vi "Connect If Necessary.vi"(8 "error in (no error)":errorcluster, 11 "Plugin in":refnum<class "Modbus.lvclass">) -> (0 "error out":errorcluster, 3 "Plugin out":refnum<class "Modbus.lvclass">)   [LabVIEW 2026, in "Modbus.lvlib" / "Modbus.lvclass"]
uses:
  Modbus.lvclass
  Modbus.lvclass/Modbus.ctl
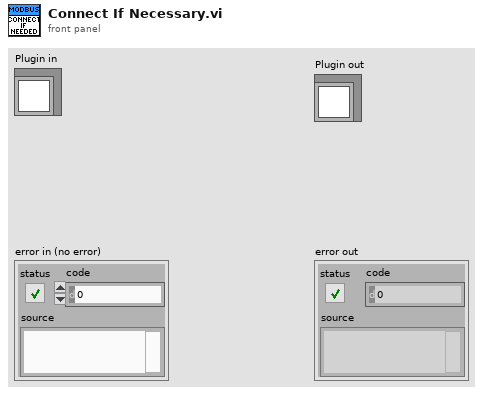
[diagram p1: front panel]
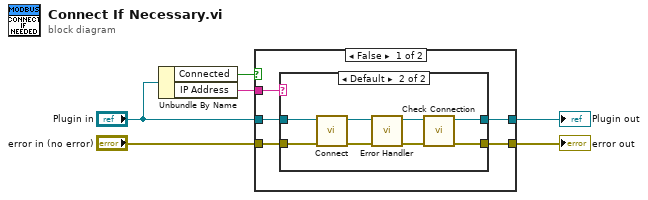
[diagram p0: block diagram]
diagram:
  n1 = Unbundle By Name("Plugin in") -> ("Connected"=w1:bool, "IP Address"=w5:string)
  n2 = case shown="False" w1 {
    tunnel: "error in (no error)" -> [w11 w23]
    tunnel: w5 -> [w10 _]
    tunnel: [w9 w23] -> w4
    tunnel: [w7 w22] -> w3
    tunnel: "Plugin in" -> [w8 w22]
    frame False {
      n3 = case shown="Default" w10 {
        tunnel: [w13 w18] -> w9
        tunnel: w11 -> [w13 w21]
        tunnel: w8 -> [w12 w17]
        tunnel: [w12 w14] -> w7
        frame "" {
          # "Don't try to connect if IP is empty"
        }
        frame Default {
          n4 = call "Connect.vi"("error in (no error)"=w21, "Modbus in"=w17) -> ("error out"=w20:errorcluster, "Modbus out"=w16:refnum<class "Modbus.lvclass">)  [unwired: 8 in]
          n5 = call "Error Handler.vi"("error in (no error)"=w20, "Modbus in"=w16) -> ("error out"=w19:errorcluster, "Modbus out"=w15:refnum<class "Modbus.lvclass">)  [unwired: 8 in]
          n6 = call "Check Connection.vi"("error in (no error)"=w19, "Plugin in"=w15) -> ("error out"=w18:errorcluster, "Plugin out"=w14:refnum<class "Modbus.lvclass">)  [unwired: 8 in]
        }
      }
    }
    frame True {
      # "Already connected"
    }
  }
  "error out" <- w4
  "Plugin out" <- w3
